vi "PostCopyScripting.vi"(10 "MetaDataObj":refnum<class "MetaDataObj.lvclass">, 11 "User Project":refnum<vi>) -> ()   [LabVIEW 2013, in "FixedChannelTBModuleDecideFeatures.lvclass"]
uses:
  FixedChannelTBModuleDecideFeatures.lvclass
  <resource>/dialog/NewProjectWizard/MetaDataObj/MetaDataObj.lvclass
  FixedChannelTBModuleDecideFeatures.lvclass/FixedChannelTBModuleDecideFeatures.ctl
  Read component name.vi
  Read Channel Specification.vi
  <vilib>/NI/DCAF/Tag Editor Core/control module/script/control module data interface generator.lvlib
  <vilib>/Utility/EditLVLibs/Edit LVLibs.lvlib
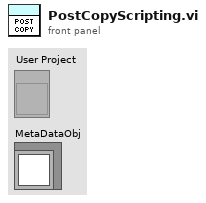
[diagram p1: front panel]
types:
  T1 = typedef "channel configuration.ctl" = cluster{"Name":string, "channel classification":T2, "data type":T3}
  T2 = typedef "TBM channel.lvclass/channel classification.ctl" = enum16{"input data", "output data", "processing parameter", "processing result"}
  T3 = typedef "tag bus.lvlib/tag descriptor.lvclass/Data Type.ctl" = enum16{"Double", "Single", "I64", "I32", "I16", "I8", "U64", "U32", "U16", "U8", "Boolean", "String", "Array of Double", "Array of Single", "Array of I64", "Array of I32", "Array of I16", "Array of I8", "Array of U64", "Array of U32", "Array of U16", "Array of U8", "Array of Boolean", "Array of String"}
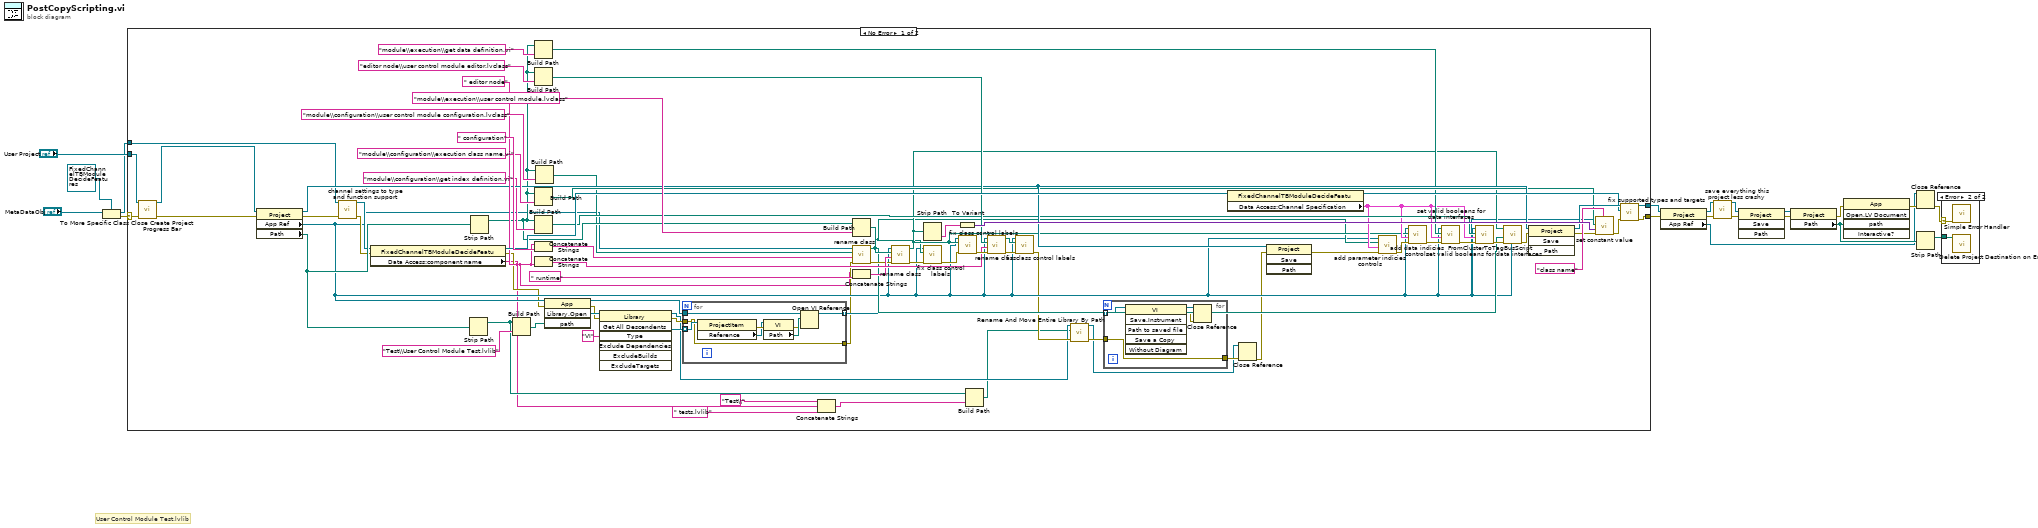
[diagram p0: block diagram]
diagram:
  # "User Control Module Test.lvlib"
  n1 = To More Specific Class(target class=refnum<class "FixedChannelTBModuleDecideFeatures.lvclass"> refnum ("DecideProjectFeatures.lvclass"), reference="MetaDataObj") -> (specific class reference=w10:refnum<class "FixedChannelTBModuleDecideFeatures.lvclass">, error out=w17:errorcluster)  [unwired: 1 in]
  n2 = case shown="No Error" w17 {
    selector: w17 -> [w60 w110]
    tunnel: [w78 w111] -> w2
    tunnel: "User Project" -> [w61 w111]
    tunnel: [w79 w110] -> w3
    tunnel: w10 -> [w65 _]
    frame No Error {
      n3 = call <resource>:"Close Create Project Progress Bar.vi"("error in (no error)"=w60, "Project"=w61) -> ("error out"=w59:errorcluster, "dup Project"=w58:refnum<vi>)  [unwired: 8 in]
      n4 = property class="Project"(reference=w58, error in=w59) -> (reference out=w69:refnum<vi>, error out=w64:errorcluster, "App Ref"=w41:refnum<vi>, "Path"=w68:path)
      n5 = call "channel settings to type and function support.vi"("error in"=w64, "FixedChannelTBModuleDecideFeatures in"=w65) -> ("error out"=w67:errorcluster, "FixedChannelTBModuleDecideFeatures out"=w66:refnum<class "FixedChannelTBModuleDecideFeatures.lvclass">)  [unwired: 8 in]
      n6 = property class="FixedChannelTBModuleDecideFeatu"(reference=w66, error in=w67) -> (reference out=w94:refnum<class "FixedChannelTBModuleDecideFeatures.lvclass">, error out=w29:errorcluster, "Data Access:component name"=w21:string)
      n7 = Strip Path(path=w68) -> (stripped path=w24:path)  [unwired: 1 out]
      n8 = Strip Path(path=w68) -> (stripped path=w55:path)  [unwired: 1 out]
      n9 = Build Path(base path=w24, name or relative path="Test\\User Control Module Test.lvlib") -> (appended path=w42:path)
      n10 = Build Path(base path=w55, name or relative path="module\\execution\\get data definition.vi") -> (appended path=w53:path)
      n11 = Build Path(base path=w55, name or relative path="editor node\\user control module editor.lvclass") -> (appended path=w85:path)
      n12 = Build Path(base path=w55, name or relative path="module\\configuration\\execution class name.vi") -> (appended path=w63:path)
      n13 = Build Path(base path=w55, name or relative path="module\\configuration\\get index definition.vi") -> (appended path=w51:path)
      n14 = Concatenate Strings(w21, " configuration" ("string")) -> (w76:string)
      n15 = Concatenate Strings(w21, " editor node" ("string")) -> (w80:string)
      n16 = Build Path(base path=w55, name or relative path="module\\configuration\\user control module configuration.lvclass") -> (appended path=w47:path)
      n17 = invoke class="App" method="Library.Open"(reference=w41, error in=w29, "path"=w42) -> (reference out=w35:refnum<vi>, error out=w37:errorcluster, "Open Library"=w40:refnum<vi>)  [unwired: 1 in, 1 out]
      n18 = invoke class="Library" method="Get All Descendents"(reference=w40, error in=w37, "Type"="VI") -> (reference out=w27:refnum<vi>, error out=w36:errorcluster, "All Descendents"=w39:refnum<vi>[])  [unwired: 4 in, 4 out]
      n19 = for {
        tunnel: w39 -> [w105] mode=indexing
        tunnel: w36 -> [w102]
        tunnel: w35 -> [w104]
        tunnel: [w103] -> w34 mode=indexing
        tunnel: [w102] -> w30
        n20 = property class="ProjectItem"(reference=w105) -> (error out=w109:errorcluster, "Reference"=w108:refnum<vi>)  [unwired: 1 in, 1 out]
        n21 = property class="VI"(reference=w108, error in=w109) -> (error out=w106:errorcluster, "Path"=w107:path)  [unwired: 1 out]
        n22 = Open VI Reference(application reference (local)=w104, vi path=w107, error in (no error)=w106) -> (vi reference=w103:refnum<vi>)  [unwired: 3 in, 1 out]
      }
      n23 = Concatenate Strings("Test\\" ("string"), w21, " tests.lvlib" ("string")) -> (w23:string)
      n24 = Build Path(base path=w55, name or relative path="module\\execution\\user control module.lvclass") -> (appended path=w46:path)
      n25 = call "rename class.vi"("error in"=w30, "new name"=w76, "class path"=w47, "Application in"=w41) -> ("error out"=w72:errorcluster, "New Library Path"=w44:path)  [unwired: 6 in]
      n26 = Concatenate Strings(w21, " runtime" ("string")) -> (w73:string)
      n27 = call "rename class.vi"("error in"=w72, "new name"=w73, "class path"=w46, "Application in"=w41) -> ("error out"=w88:errorcluster, "New Library Path"=w45:path)  [unwired: 6 in]
      n28 = Strip Path(path=w45) -> (name=w75:string)  [unwired: 1 out]
      n29 = call "fix class control labels.vi"("error in"=w88, "class to load"=w44, "Application in"=w41) -> ("error out"=w87:errorcluster)  [unwired: 8 in]
      n30 = To Variant(anything=w75) -> (Variant=w93:variant)
      n31 = call "fix class control labels.vi"("error in"=w87, "class to load"=w45, "Application in"=w41) -> ("error out"=w82:errorcluster)  [unwired: 8 in]
      n32 = Build Path(base path=w24, name or relative path=w23) -> (appended path=w25:path)
      n33 = call "rename class.vi"("error in"=w82, "new name"=w80, "class path"=w85, "Application in"=w41) -> ("error out"=w83:errorcluster, "New Library Path"=w84:path)  [unwired: 6 in]
      n34 = call "fix class control labels.vi"("error in"=w83, "class to load"=w84, "Application in"=w41) -> ("error out"=w28:errorcluster)  [unwired: 8 in]
      n35 = call <vilib>:"Rename And Move Entire Library By Path.vi"("error in (no error)"=w28, "New library path"=w25, "Library ref in"=w27) -> ("error out"=w33:errorcluster, "Library ref out"=w26:refnum<vi>)  [unwired: 7 in]
      n36 = for {
        tunnel: w34 -> [w99] mode=indexing
        tunnel: [w98] -> w32
        tunnel: w33 -> [w98]
        n37 = invoke class="VI" method="Save.Instrument"(reference=w99) -> (reference out=w100:refnum<vi>, error out=w101:errorcluster)  [unwired: 5 in, 4 out]
        n38 = Close Reference(reference=w100, error in (no error)=w101) -> ()  [unwired: 1 out]
      }
      n39 = property class="FixedChannelTBModuleDecideFeatu"(reference=w94) -> (reference out=w71:refnum<class "FixedChannelTBModuleDecideFeatures.lvclass">, "Data Access:Channel Specification"=w50:T1[])  [unwired: 1 in, 1 out]
      n40 = Close Reference(reference=w26, error in (no error)=w32) -> (error out=w31:errorcluster)
      n41 = invoke class="Project" method="Save"(reference=w69, error in=w31) -> (error out=w70:errorcluster)  [unwired: 2 in, 3 out]
      n42 = call "add parameter indicies controls.vi"("error in"=w70, "Channels to create"=w50, "cfg class path"=w44, "Application in"=w41) -> ("error out"=w62:errorcluster)  [unwired: 7 in]
      n43 = call "add data indicies controls.vi"("error in"=w62, "Channels to create"=w50, "runtime class path"=w45, "Application in"=w41) -> ("error out"=w54:errorcluster)  [unwired: 7 in]
      n44 = call "set valid booleans for data interfaces.vi"("error in"=w54, "Channel Specification"=w50, "vi path"=w53, "Application in"=w41) -> ("error out"=w52:errorcluster)  [unwired: 7 in]
      n45 = call "set valid booleans for data interfaces.vi"("error in"=w52, "Channel Specification"=w50, "vi path"=w51, "Application in"=w41) -> ("error out"=w49:errorcluster)  [unwired: 7 in]
      n46 = call <vilib>:"FromClusterToTagBusScript.vi"("application reference (local)"=w41, "error in"=w49, "configuration class path"=w44, "runtime class path"=w45) -> ("error out"=w48:errorcluster)  [unwired: 7 in]
      n47 = invoke class="Project" method="Save"(reference=w69, error in=w48) -> (reference out=w89:refnum<vi>, error out=w90:errorcluster)  [unwired: 2 in, 2 out]
      n48 = call "set constant value.vi"("control name"="class name", "error in"=w90, "data to set"=w93, "vi path"=w63, "Application in"=w41) -> ("error out"=w77:errorcluster)  [unwired: 6 in]
      n49 = call "fix supported types and targets.vi"("error in"=w77, "DecideProjectFeatures in"=w71, "User Project in"=w89) -> ("error out"=w79:errorcluster, "User Project out"=w78:refnum<vi>)  [unwired: 7 in]
    }
    frame Error {
    }
  }
  n50 = property class="Project"(reference=w2, error in=w3) -> (reference out=w7:refnum<vi>, error out=w8:errorcluster, "App Ref"=w1:refnum<vi>)
  n51 = call "save everything this project less crashy.vi"("error in"=w8, "Project in"=w7) -> ("error out"=w4:errorcluster, "Project out"=w9:refnum<vi>)  [unwired: 8 in]
  n52 = invoke class="Project" method="Save"(reference=w9, error in=w4) -> (reference out=w13:refnum<vi>, error out=w14:errorcluster)  [unwired: 2 in, 2 out]
  n53 = property class="Project"(reference=w13, error in=w14) -> (error out=w16:errorcluster, "Path"=w11:path)  [unwired: 1 out]
  n54 = invoke class="App" method="Open.LV Document"(error in=w16, "path"=w11) -> (error out=w15:errorcluster)  [unwired: 3 in, 4 out]
  n55 = Close Reference(reference=w1, error in (no error)=w15) -> (error out=w6:errorcluster)
  n56 = Strip Path(path=w11) -> (stripped path=w5:path)  [unwired: 1 out]
  n57 = case shown="Error" w6 {
    selector: w6 -> [_ w112]
    tunnel: w5 -> [_ w113]
    frame No Error {
    }
    frame Error {
      n58 = call <vilib>:"Simple Error Handler.vi"("error in (no error)"=w112) -> ()  [unwired: 4 in, 5 out]
      n59 = call <resource>:"Delete Project Destination on Error.vi"("Project Destination Root"=w113) -> ()  [unwired: 11 in]
    }
  }
